vi "Create PV Data.vi"(8 "error in (no error)":errorcluster, 11 "NT Scalar (Numeric) in":refnum<class "NT Scalar (Numeric).lvclass">) -> (0 "error out":errorcluster, 2 "PV Data out":refnum<class "PV Data.lvclass">, 3 "NT Scalar (Numeric) out":refnum<class "NT Scalar (Numeric).lvclass">)   [LabVIEW 2020, in "PV Access.lvlib" / "PV Data.lvlib" / "NT Scalar (Numeric).lvclass"]
uses:
  NT Scalar (Numeric).lvclass
  PV Data/PV Data.lvclass
  Error Codes.ctl
  PV Data.lvlib
  Value Fields.ctl
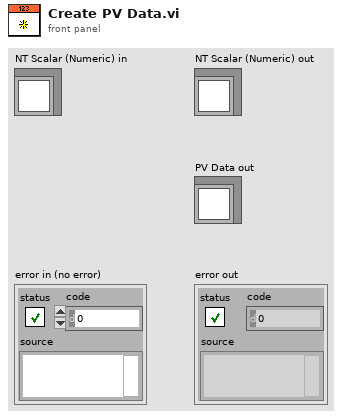
[diagram p1: front panel]
types:
  T1 = typedef "PV Access.lvlib/PV Data.lvlib/Value Fields.ctl" = cluster{"Display":bool, "Control":bool, "Alarm Limits":bool}
  T2 = typedef "PV Access.lvlib/PV Data.lvlib/Error Codes.ctl" = i32
  T3 = typedef "PV Access.lvlib/PV Data.lvlib/Type Code.ctl" = enum8{"Null", "Bool", "BoolA", "Int8", "Int8A", "Int16", "Int16A", "Int32", "Int32A", "Int64", "Int64A", "UInt8", "UInt8A", "UInt16", "UInt16A", "UInt32", "UInt32A", "UInt64", "UInt64A", "Float32", "Float32A", "Float64", "Float64A", "String", "StringA", "Struct", "StructA", "Union", "UnionA", "Any", "AnyA"}
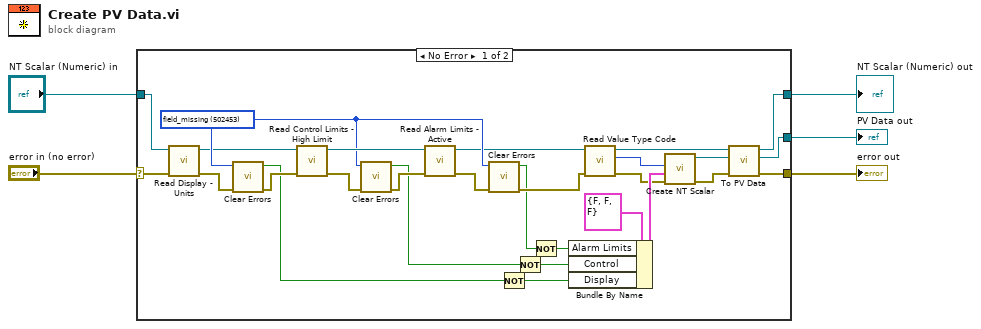
[diagram p0: block diagram]
diagram:
  n1 = case shown="No Error" "error in (no error)" {
    selector: "error in (no error)" -> [w26 w35]
    tunnel: [w31 w35] -> w4
    tunnel: [w13 w34] -> w1
    tunnel: "NT Scalar (Numeric) in" -> [w27 w34]
    tunnel: [w30 _] -> w3
    frame No Error {
      w20 = T2 502453 items=["unspecified"=502450, "interrupted"=502451, "timeout"=502452, "field_missing"=502453, "cannot_convert_value"=502454, "type_mismatch"=502455] ("Ring")
      n2 = call-dynamic "Read Display - Units.vi"("error in (no error)"=w26, "NT Scalar (Numeric) in"=w27) -> ("error out"=w25:errorcluster, "NT Scalar (Numeric) out"=w6:refnum<class "NT Scalar (Numeric).lvclass">)  [unwired: 7 in, 1 out]
      n3 = call <vilib>:"Clear Errors.vi"("error in (no error)"=w25, "specific error code to clear (0: all)"=w20) -> ("error out"=w23:errorcluster, "specific error cleared?"=w12:bool)  [unwired: 4 in]
      n4 = call-dynamic "Read Control Limits - High Limit.vi"("error in (no error)"=w23, "NT Scalar (Numeric) in"=w6) -> ("error out"=w22:errorcluster, "NT Scalar (Numeric) out"=w24:refnum<class "NT Scalar (Numeric).lvclass">)  [unwired: 7 in, 1 out]
      n5 = call <vilib>:"Clear Errors.vi"("error in (no error)"=w22, "specific error code to clear (0: all)"=w20) -> ("error out"=w21:errorcluster, "specific error cleared?"=w9:bool)  [unwired: 4 in]
      n6 = call-dynamic "Read Alarm Limits - Active.vi"("error in (no error)"=w21, "NT Scalar (Numeric) in"=w24) -> ("error out"=w29:errorcluster, "NT Scalar (Numeric) out"=w18:refnum<class "NT Scalar (Numeric).lvclass">)  [unwired: 7 in, 1 out]
      n7 = call <vilib>:"Clear Errors.vi"("error in (no error)"=w29, "specific error code to clear (0: all)"=w20) -> ("error out"=w17:errorcluster, "specific error cleared?"=w8:bool)  [unwired: 4 in]
      n8 = Not(x=w12) -> (.not. x?=w11:bool)
      n9 = Not(x=w9) -> (.not. x?=w10:bool)
      n10 = Not(x=w8) -> (.not. x?=w7:bool)
      n11 = Bundle By Name(cluster=T1 {"Display"=FALSE, "Control"=FALSE, "Alarm Limits"=FALSE} ("Value fields"), "Alarm Limits"=w7, "Control"=w10, "Display"=w11) -> (w19:T1)
      n12 = call-dynamic "Read Value Type Code.vi"("error in (no error)"=w17, "NT Scalar in"=w18) -> ("error out"=w15:errorcluster, "type code"=w16:T3, "NT Scalar out"=w14:refnum<class "NT Scalar (Numeric).lvclass">)  [unwired: 7 in]
      n13 = call "Create NT Scalar.vi"("error in"=w15, "value fields"=w19, "type code"=w16) -> ("error out"=w32:errorcluster, "PV Data out"=w33:refnum<class "PV Data.lvclass">)  [unwired: 7 in]
      n14 = call-dynamic "To PV Data.vi"("error in"=w32, "PV data in"=w33, "Base Interface in"=w14) -> ("error out"=w31:errorcluster, "PV data out"=w30:refnum<class "PV Data.lvclass">, "Base Interface out"=w13:refnum<class "NT Scalar (Numeric).lvclass">)  [unwired: 6 in]
    }
    frame Error {
    }
  }
  "NT Scalar (Numeric) out" <- w1
  "error out" <- w4
  "PV Data out" <- w3
